vi "Encode Parameter and Update Word (32-bit).vi"(8 "error in":errorcluster, 9 "parameter definition":T1={"start index"=10, "size"=19, "encoding"=enum."BNR", "signed"=FALSE, "scale multiplier"=1.0, "scale offset"=0.0}, 10 "parameter value":dbl, 11 "word in":u32 format="%032b") -> (0 "error out":errorcluster, 3 "word out":u32 format="%032b")   [LabVIEW 2020]
uses:
  Parameter Definition.ctl
  <vilib>/NI/NI VeriStand Encoding and Decoding/Encoding.ctl
  <vilib>/NI/NI VeriStand Encoding and Decoding/Parity.ctl
  1445f95d-237d-4fc6-96b9-8992d347f513.vi
  6b8853f0-8e5d-49e3-9391-4d3f8e5314b0.vi
  2babc4f4-546e-4d35-846d-a4a1fbac0249.vi
  1445f95d-237d-4fc6-96b9-8992d347f513.vi/9377bb8f-44b5-4a8f-87f1-966fd5a9edcc.vi
  1445f95d-237d-4fc6-96b9-8992d347f513.vi/e95d9d1f-307c-44d6-9f26-c3f519a4990d.vi
  1445f95d-237d-4fc6-96b9-8992d347f513.vi/0c23f515-4369-4514-bc3d-4444e6b437b2.vi
  6b8853f0-8e5d-49e3-9391-4d3f8e5314b0.vi/136dcdcb-2dd3-4a4d-a796-a8f7a3f8e1ac.vi
  6b8853f0-8e5d-49e3-9391-4d3f8e5314b0.vi/a54b505c-1216-4ef4-8378-3ceda9d188df.vi
  <vilib>/NI/NI VeriStand Encoding and Decoding/Get Bits Per Digit from Base.vi
  <vilib>/NI/NI VeriStand Encoding and Decoding/Encoding and Decoding.lvlib
panel:
  # "P (1) | SSM (2) | Parameter (19) | SDI (2) | LABEL (8)"
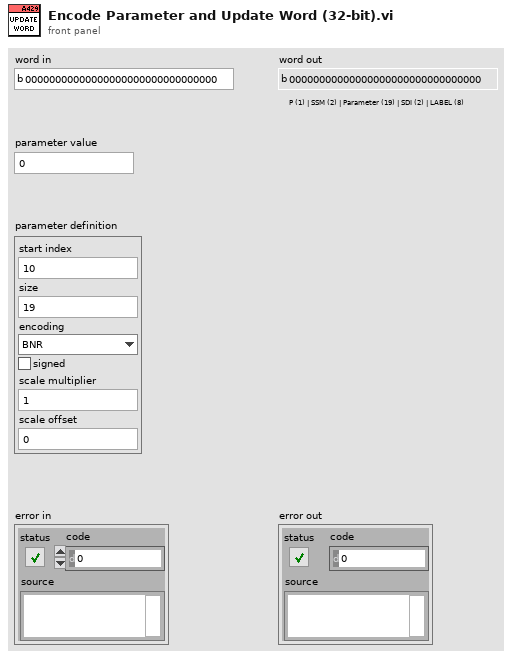
[diagram p1: front panel]
types:
  T1 = typedef "Parameter Definition.ctl" = cluster{"start index":i32, "size":i32, "encoding":T2, "signed":bool, "scale multiplier":dbl, "scale offset":dbl}
  T2 = typedef "Encoding and Decoding.lvlib/Encoding.ctl" = enum16{"BNR", "BCD", "Discrete"}
  T3 = typedef "Encoding and Decoding.lvlib/Parity.ctl" = enum16{"Even", "Odd"}
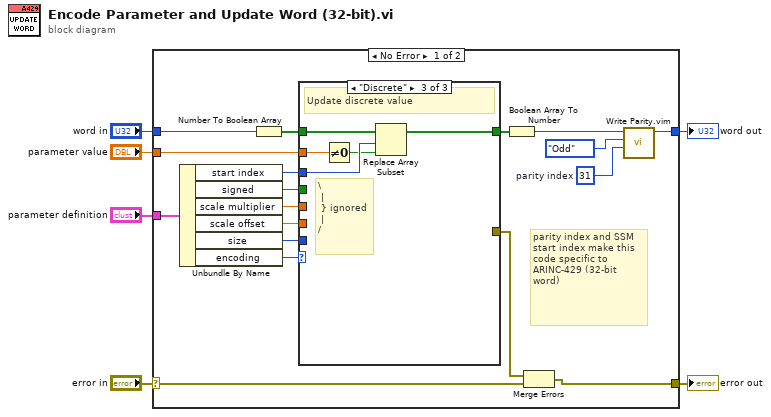
[diagram p0: block diagram]
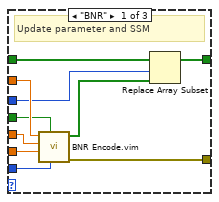
[diagram p2: hidden frame]
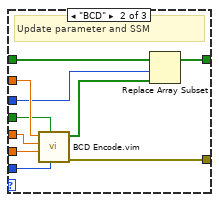
[diagram p3: hidden frame]
diagram:
  n1 = case shown="No Error" "error in" {
    selector: "error in" -> [w13 w50]
    tunnel: "parameter value" -> [w17 _]
    tunnel: "word in" -> [w16 w51]
    tunnel: "parameter definition" -> [w15 _]
    tunnel: [w8 w51] -> w3
    tunnel: [w12 w50] -> w1
    frame No Error {
      w7 = 31  # parity index
      # "parity index and SSM start index make this code specific to ARINC-429 (32-bit word)"
      n2 = Unbundle By Name(w15) -> ("start index"=w18:i32, "signed"=w19:bool, "scale multiplier"=w22:dbl, "scale offset"=w21:dbl, "size"=w20:i32, "encoding"=w24:T2)
      n3 = Number To Boolean Array(number=w16) -> (Boolean array=w23:bool[])
      n4 = case shown="\"Discrete\"" w24 {
        tunnel: w17 -> [w34 w44 w49]
        tunnel: w22 -> [w33 w43 _]
        tunnel: w21 -> [w32 w42 _]
        tunnel: w20 -> [w31 w40 _]
        tunnel: w19 -> [w25 w41 _]
        tunnel: [w30 w39 _] -> w14
        tunnel: w18 -> [w28 w37 w48]
        tunnel: w23 -> [w27 w38 w46]
        tunnel: [w26 w35 w45] -> w10
        frame "BNR" {
          # "Update parameter and SSM"
          n5 = call "BNR Encode.vim"("data size (bits)"=w31, "signed"=w25, "scale offset"=w32, "scale multiplier"=w33, "value"=w34) -> ("error out"=w30:errorcluster, "BNR encoded value"=w29:bool[])  [unwired: 5 in]
          n6 = Replace Array Subset(array=w27, new element=w29, index=w28) -> (w26:bool[])
        }
        frame "BCD" {
          # "Update parameter and SSM"
          n7 = call "BCD Encode.vim"("data size (bits)"=w40, "signed"=w41, "scale offset"=w42, "scale multiplier"=w43, "value"=w44) -> ("error out"=w39:errorcluster, "BCD encoded value"=w36:bool[])  [unwired: 4 in, 1 out]
          n8 = Replace Array Subset(array=w38, new element=w36, index=w37) -> (w35:bool[])
        }
        frame "Discrete" {
          # "\\\n |\n } ignored \n |\n/"
          # "Update discrete value"
          n9 = Not Equal To 0?(x=w49) -> (x != 0?=w47:bool)
          n10 = Replace Array Subset(array=w46, new element=w47, index=w48) -> (w45:bool[])
        }
      }
      n11 = Boolean Array To Number(Boolean array=w10) -> (number=w9:u32)
      n12 = Merge Errors(w14, w13) -> (w12:errorcluster)
      n13 = call "Write Parity.vim"("parity index"=w7, "parity"=Parity."Odd", "word in"=w9) -> ("word out"=w8:u32)  [unwired: 8 in]
    }
    frame Error {
    }
  }
  "word out" <- w3
  "error out" <- w1
